vi "ZM-ROOT-showError.vi"(8 "error in (no error)":errorcluster, 10 "package":refnum<class "ZM-PC-package.lvclass">, 11 "ZM-ROOT-root in":refnum<class "ZM-ROOT-root.lvclass">) -> (0 "error out":errorcluster, 3 "ZM-ROOT-root out":refnum<class "ZM-ROOT-root.lvclass">)   [LabVIEW 2020, in "ZM-ROOT-root.lvlib" / "ZM-ROOT-root.lvclass"]
doc: "Shows an error package on the root's panel: fires the error user event with the package's JSON, which ZM-ROOT-helperPanel appends to errors. If the sender is the CM, it sets cmRunning = FALSE, so nothing more is forwarded to it."
uses:
  ZM-ROOT-root.lvclass
  common/ZM-PC-packages/ZM-PC-package/ZM-PC-package.lvclass
  common/ZM-PC-packages/ZM-PC-EP-error_package/ZM-PC-EP-error_package.lvclass
  ZM-ROOT-root.lvclass/ZM-ROOT-root.ctl
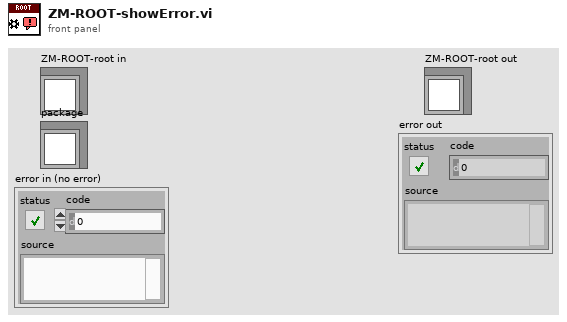
[diagram p1: front panel]
types:
  T1 = typedef "ZM-ROOT-root.lvlib/ZM-ROOT-root.lvclass/ZM-ROOT-EVENTS.ctl" = cluster{"stop":refnum<user-event>, "error":refnum<user-event>}
  T2 = typedef "ZM-PC-packages.lvlib/ZM-PC-EP-error_package.lvclass/ZM-PC-EP-DATA.ctl" = cluster{"sender":string, "code":i32, "source":string}
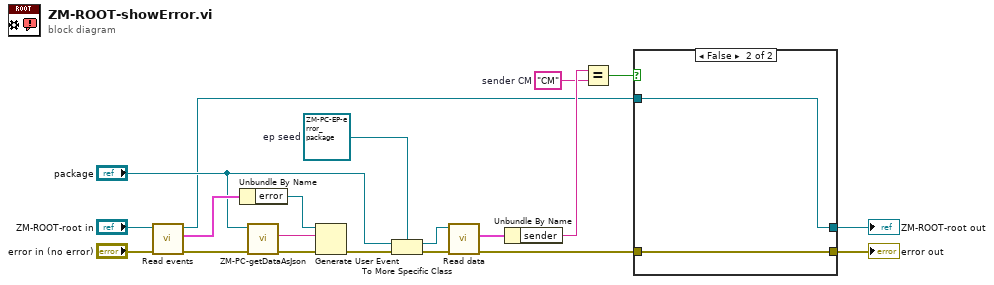
[diagram p0: block diagram]
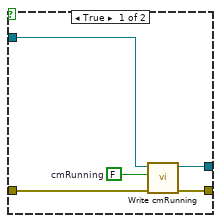
[diagram p2: hidden frame]
diagram:
  w6 = "CM"  # sender CM
  w11 = refnum<class "ZM-PC-EP-error_package.lvclass"> refnum  # ep seed
  n1 = call "Read events.vi"("error in (no error)"="error in (no error)", "ZM-ROOT-root in"="ZM-ROOT-root in") -> ("error out"=w17:errorcluster, "ZM-ROOT-EVENTS"=w18:T1, "ZM-ROOT-root out"=w5:refnum<class "ZM-ROOT-root.lvclass">)  [unwired: 7 in]
  n2 = Unbundle By Name(w18) -> ("error"=w16:refnum<user-event>)
  n3 = call-dynamic "ZM-PC-getDataAsJson.vi"("error in (no error)"=w17, "ZM-PC-package in"="package") -> ("error out"=w14:errorcluster, "json"=w15:string)  [unwired: 7 in, 1 out]
  n4 = Generate User Event(user event=w16, event data cluster=w15, error in=w14) -> (error out=w12:errorcluster)  [unwired: 1 in, 1 out]
  n5 = To More Specific Class(target class=w11, reference="package", error in=w12) -> (specific class reference=w9:refnum<class "ZM-PC-EP-error_package.lvclass">, error out=w10:errorcluster)
  n6 = call "Read data.vi"("error in (no error)"=w10, "ZM-PC-EP-error_package in"=w9) -> ("error out"=w4:errorcluster, "ZM-PC-EP-DATA"=w8:T2)  [unwired: 7 in, 1 out]
  n7 = Unbundle By Name(w8) -> ("sender"=w7:string)
  n8 = Equal?(x=w7, y=w6) -> (x = y?=w3:bool)
  n9 = case shown="False" w3 {
    tunnel: w5 -> [w24 w27]
    tunnel: w4 -> [w25 w26]
    tunnel: [w22 w27] -> w2
    tunnel: [w21 w26] -> w1
    frame True {
      w23 = FALSE  # cmRunning
      n10 = call "Write cmRunning.vi"("error in (no error)"=w25, "cmRunning"=w23, "ZM-ROOT-root in"=w24) -> ("error out"=w21:errorcluster, "ZM-ROOT-root out"=w22:refnum<class "ZM-ROOT-root.lvclass">)  [unwired: 7 in]
    }
    frame False {
    }
  }
  "ZM-ROOT-root out" <- w2
  "error out" <- w1
